vi "Generate_Model_Info(CSV).vi"(11 "Model_Info_and_Report":T1={"Idx"=0, "Name"="", "Feature Extractor"="wrn_50_2_2_bnmerge", "Layers"="", "DS_Size"=0, "H"=0, "W"=0, "Coreset Size"=0, "Proj_Dim"=0, "Good_Max(Img)"=0.0, "Bad_Min(Img)"=0.0, "Rel_Margin"=0.0, "Image_AUC"=0.0, "Pixel_AUC"=0.0, "Image_F1_Max"=0.0, "Pixel_F1_Max"=0.0, "Train_Time"=0.0, "Inf_Time"=0.0} {"Rel_Margin" format="%#.5f"; "Bad_Min(Img)" format="%#.5f"; "Good_Max(Img)" format="%#.5f"; "Pixel_F1_Max" format="%#.5f"; "Pixel_AUC" format="%#.5f"; "Image_F1_Max" format="%#.5f"; "Image_AUC" format="%#.5f"}) -> (3 "Model_Info(CSV)":string)   [LabVIEW 2020]
uses:
  Controls/Model_Info_and_Report.ctl
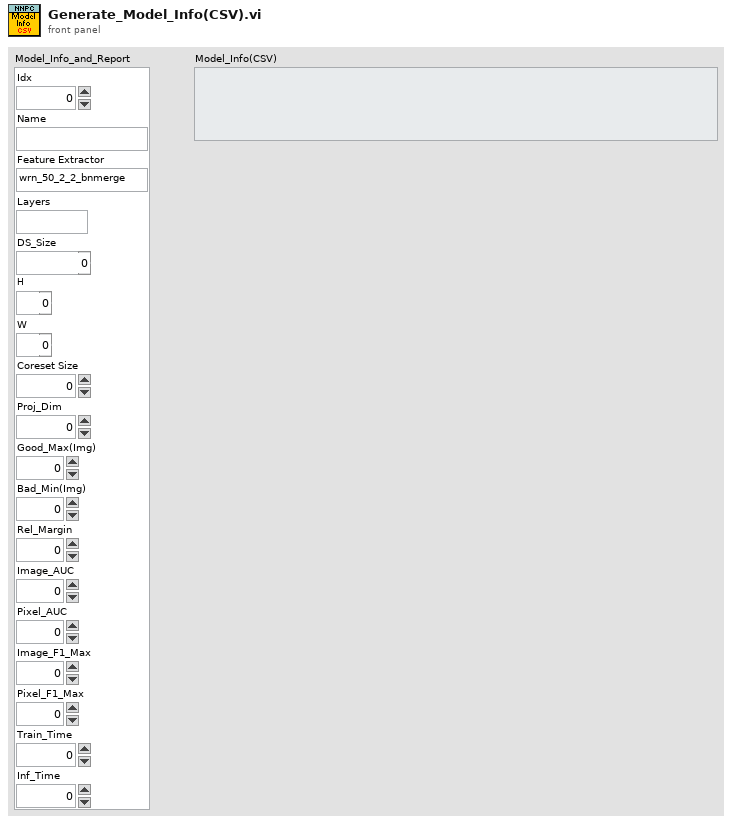
[diagram p1: front panel]
types:
  T1 = typedef "Model_Info_and_Report.ctl" = cluster{"Idx":i32, "Name":string, "Feature Extractor":string, "Layers":string, "DS_Size":i32, "H":i32, "W":i32, "Coreset Size":i32, "Proj_Dim":i32, "Good_Max(Img)":sgl, "Bad_Min(Img)":sgl, "Rel_Margin":sgl, "Image_AUC":sgl, "Pixel_AUC":sgl, "Image_F1_Max":sgl, "Pixel_F1_Max":sgl, "Train_Time":dbl, "Inf_Time":dbl}
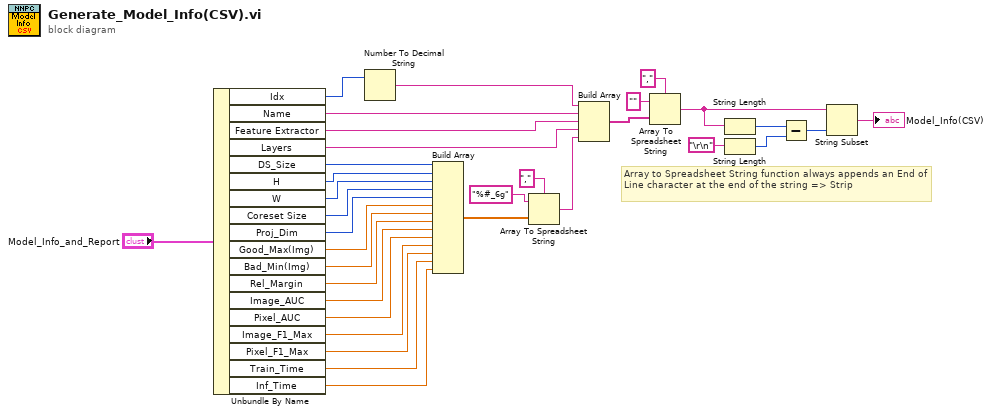
[diagram p0: block diagram]
diagram:
  # "Array to Spreadsheet String function always appends an End of Line character at the end of the string => Strip"
  n1 = Unbundle By Name("Model_Info_and_Report") -> ("Idx"=w18:i32, "Name"=w13:string, "Feature Extractor"=w12:string, "Layers"=w1:string, "DS_Size"=w19:i32, "H"=w20:i32, "W"=w23:i32, "Coreset Size"=w33:i32, "Proj_Dim"=w25:i32, "Good_Max(Img)"=w21:sgl, "Bad_Min(Img)"=w22:sgl, "Rel_Margin"=w16:sgl, "Image_AUC"=w27:sgl, "Pixel_AUC"=w28:sgl, "Image_F1_Max"=w29:sgl, "Pixel_F1_Max"=w30:sgl, "Train_Time"=w31:dbl, "Inf_Time"=w24:dbl)
  n2 = Number To Decimal String(number=w18) -> (decimal integer string=w14:string)  [unwired: 1 in]
  n3 = Build Array(w19, w20, w23, w33, w25, w21, w22, w16, w27, w28, w29, w30, w31, w24) -> (w32:dbl[])
  n4 = Array To Spreadsheet String(delimiter (Tab)=",", array=w32, 3:"%#_6g" ("spreadsheet string")) -> (spreadsheet string=w11:string)
  n5 = Build Array(w14, w13, w12, w1, w11) -> (w9:string[])
  n6 = Array To Spreadsheet String(delimiter (Tab)=",", array=w9, 3:"" ("format string")) -> (spreadsheet string=w3:string)
  n7 = String Length(string=w3) -> (length=w6:i32)
  n8 = String Length(string="\r\n") -> (length=w5:i32)
  n9 = Subtract(x=w6, y=w5) -> (x-y=w4:i32)
  n10 = String Subset(string=w3, length (rest)=w4) -> (substring=→"Model_Info(CSV)":string)  [unwired: 1 in]
